vi "generateTempFile.vi"(8 "error in (no error)":errorcluster, 11 "MS-Excel in":refnum<class "MS-Excel.lvclass">) -> (0 "error out":errorcluster, 2 "Temporary File Path":path, 3 "MS-Excel out":refnum<class "MS-Excel.lvclass">)   [LabVIEW 2017, in "LabVIEW NPOI.lvlib" / "MS-Excel.lvclass"]
uses:
  MS-Excel.lvclass
  9e7235be-b1ca-40b6-9cb6-9008c29a5685.vi
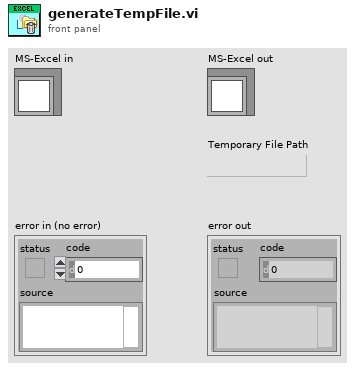
[diagram p1: front panel]
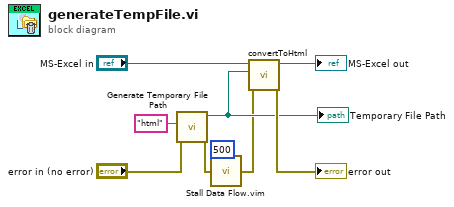
[diagram p0: block diagram]
diagram:
  n1 = call <vilib>:"Generate Temporary File Path.vi"("error in (no error)"="error in (no error)", "Temporary File Extension (tmp)"="html") -> ("error out"=w6:errorcluster, "Unique Temporary File Path"=w3:path)  [unwired: 8 in]
  "Temporary File Path" <- w3
  n2 = call "Stall Data Flow.vim"("value in"=w6, "milliseconds to wait"=u32 500) -> ("value out"=w2:errorcluster)  [unwired: 1 out]
  n3 = call-dynamic "convertToHtml.vi"("error in (no error)"=w2, "HTML File Path"=w3, "MS-Excel in"="MS-Excel in") -> ("error out"=→"error out":errorcluster, "MS-Excel out"=→"MS-Excel out":refnum<class "MS-Excel.lvclass">)  [unwired: 7 in]
